vi "Build New Ballard ARINC 429 Custom Device.vi"(7 "Base System Definition File":path=path "Support/Base.nivssdf", 10 "Hardware Configuration File":path=path "Support/Multichannel Tx and Rx HW.xml", 11 "Output System Definition File":path=path "Support/Scripted Ballard ARINC 429.nivssdf") -> (3 "Ballard ARINC 429 System Definition":path)   [LabVIEW 2020]
doc: "Overview: Demonstrates using the Ballard ARINC 429 scripting API to configure the custom device by building from configuration clusters. \n\nInstructions:\n1. Specify the Hardware Configuration File. The hardware configuration file must be consistent with the schema installed by the Ballard hardware driver at C:\\Program Files (x86)\\Astronics Ballard Technology LabVIEW Driver\\Help\\index.html. The hardware configuration file must also be consistent with the configuration in this example VI.\n2. (VeriStand) Optionally, you may open the Output System Definition File in VeriStand, configure the Target, and deploy the scripted system definition to perform avionics bus communications with Ballard ARINC 429 hardware."
uses:
  Ballard ARINC 429 Scripting Examples.lvlib
  <vilib>/addons/VeriStand Custom Device Scripting APIs/Ballard ARINC 429/Scripting/Ballard/Ballard ARINC 429 Scripting.lvlib
  <vilib>/addons/VeriStand Custom Device Scripting APIs/Ballard ARINC 429/Shared/Direction.ctl
  <vilib>/addons/VeriStand Custom Device Scripting APIs/Ballard ARINC 429/Shared/Ballard ARINC 429 Shared.lvlib
  <vilib>/addons/VeriStand Custom Device Scripting APIs/Ballard ARINC 429/Shared/SDI.ctl
  <vilib>/addons/VeriStand Custom Device Scripting APIs/Ballard ARINC 429/Shared/Transfer Type.ctl
  <vilib>/NI/NI VeriStand Encoding and Decoding/Encoding.ctl
  <vilib>/NI/NI VeriStand Encoding and Decoding/Encoding and Decoding.lvlib
  <vilib>/addons/VeriStand Custom Device Scripting APIs/Ballard ARINC 429/Shared/Parameter Definition.ctl
  NationalInstruments.VeriStand.SystemDefinitionAPI
  <vilib>/addons/VeriStand Custom Device Scripting APIs/Ballard ARINC 429/Shared/Initialization Method.ctl
  <vilib>/addons/VeriStand Custom Device Scripting APIs/Ballard ARINC 429/Shared/Device Parameters.ctl
panel:
  # "Overview: Demonstrates using the Ballard ARINC 429 scripting API to configure the custom device by building from configuration clusters. \n\nInstructions:\n1. Specify the Hardware Configuration File. The hardware configuration file must be consistent with the schema installed by the Ballard hardware driver at C:\\Program Files (x86)\\Astronics Ballard Technology LabVIEW Driver\\Help\\index.html. The hardware configuration file must also be consistent with the configuration in this example VI.\n2. (VeriStand) Optionally, you may open the Output System Definition File in VeriStand, configure the Target, and deploy the scripted system definition to perform avionics bus communications with Ballard ARINC 429 hardware."
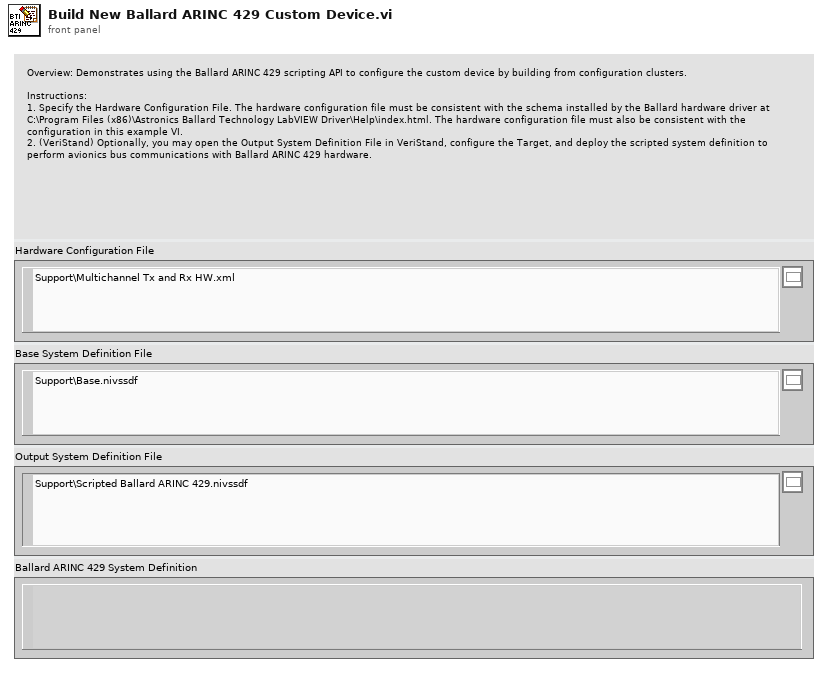
[diagram p1: front panel]
types:
  T1 = typedef "Ballard ARINC 429 Shared.lvlib/Device Parameters.ctl" = cluster{"initialization method":T2, "card number":i32, "PXI slot number":i32, "core number":i32, "core serial number":i32}
  T2 = typedef "Ballard ARINC 429 Shared.lvlib/Initialization Method.ctl" = enum16{"PXI Slot Number", "Card Number", "Core Serial Number"}
  T3 = cluster{"name":string, "unit":string, "default value":dbl}[]
  T4 = typedef "Ballard ARINC 429 Shared.lvlib/Parameter Definition.ctl" = cluster{"start index":i32, "size":i32, "encoding":T5, "signed":bool, "scale multiplier":dbl, "scale offset":dbl}
  T5 = typedef "Encoding and Decoding.lvlib/Encoding.ctl" = enum16{"BNR", "BCD", "Discrete"}
  T6 = typedef "Ballard ARINC 429 Shared.lvlib/Direction.ctl" = enum16{"Rx", "Tx"}
  T7 = typedef "Ballard ARINC 429 Shared.lvlib/Transfer Type.ctl" = enum16{"Scheduled", "Acyclic", "Block", "Strobe"}
  T8 = typedef "Ballard ARINC 429 Shared.lvlib/SDI.ctl" = i32
  T9 = typedef "Custom Device API.lvlib/Custom Device Item Ref.ctl" = u64
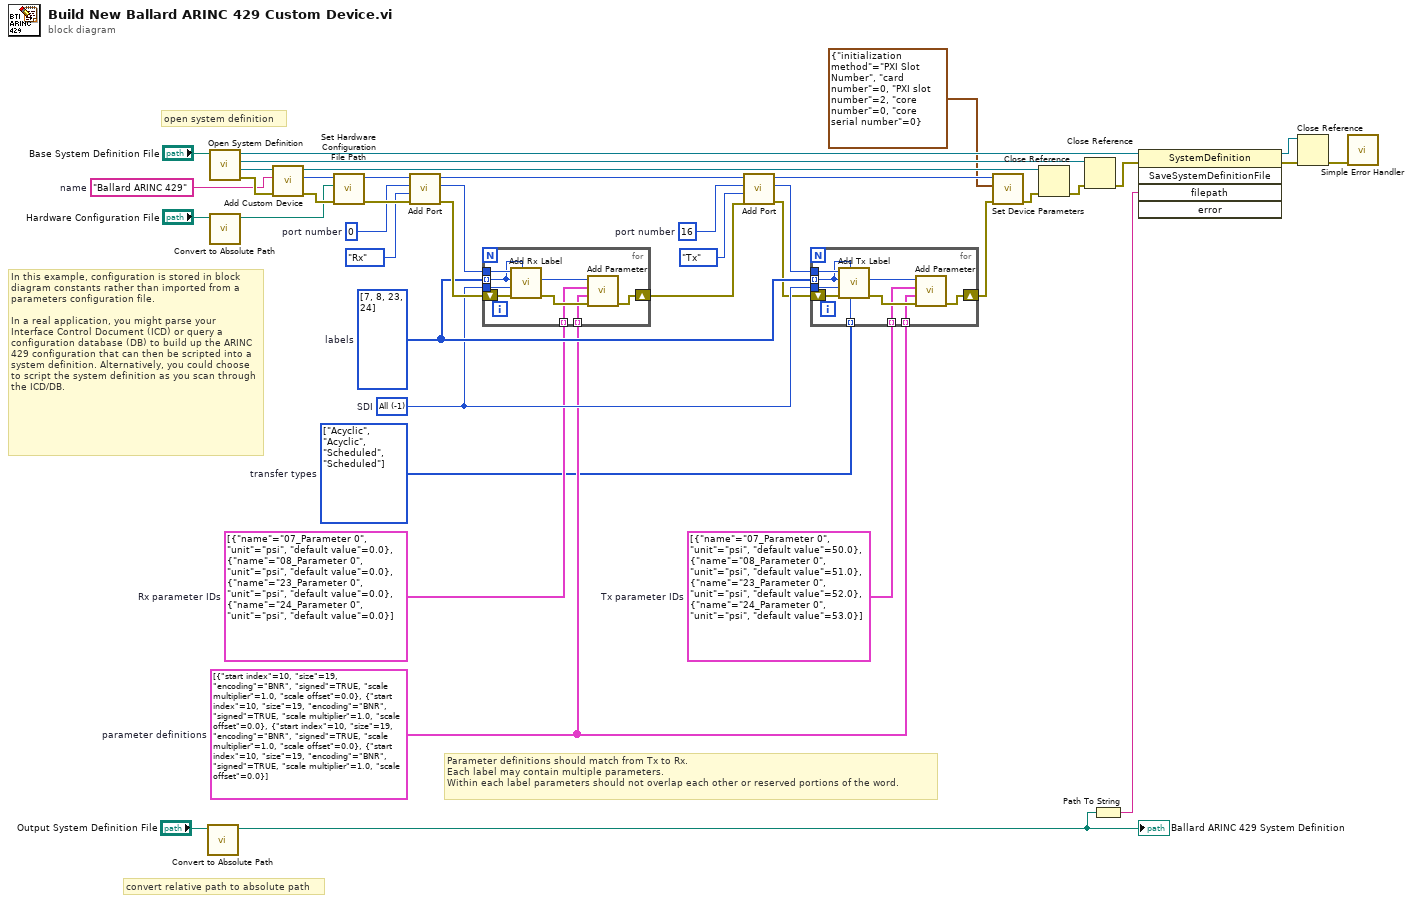
[diagram p0: block diagram]
diagram:
  w6 = T3 [{"name"="07_Parameter 0", "unit"="psi", "default value"=50.0}, {"name"="08_Parameter 0", "unit"="psi", "default value"=51.0}, {"name"="23_Parameter 0", "unit"="psi", "default value"=52.0}, {"name"="24_Parameter 0", "unit"="psi", "default value"=53.0}]  # Tx parameter IDs
  w8 = T4[] [{"start index"=10, "size"=19, "encoding"=enum."BNR", "signed"=TRUE, "scale multiplier"=1.0, "scale offset"=0.0}, {"start index"=10, "size"=19, "encoding"=enum."BNR", "signed"=TRUE, "scale multiplier"=1.0, "scale offset"=0.0}, {"start index"=10, "size"=19, "encoding"=enum."BNR", "signed"=TRUE, "scale multiplier"=1.0, "scale offset"=0.0}, {"start index"=10, "size"=19, "encoding"=enum."BNR", "signed"=TRUE, "scale multiplier"=1.0, "scale offset"=0.0}]  # parameter definitions
  w9 = T3 [{"name"="07_Parameter 0", "unit"="psi", "default value"=0.0}, {"name"="08_Parameter 0", "unit"="psi", "default value"=0.0}, {"name"="23_Parameter 0", "unit"="psi", "default value"=0.0}, {"name"="24_Parameter 0", "unit"="psi", "default value"=0.0}]  # Rx parameter IDs
  w17 = u16 16  # port number
  w7 = T7[] [enum."Acyclic", enum."Acyclic", enum."Scheduled", enum."Scheduled"] items=["Scheduled", "Acyclic", "Block", "Strobe"]  # transfer types
  w11 = T8 -1 items=["All"=-1, "0 (b00)"=0, "1 (b01)"=1, "2 (b10)"=2, "3 (b11)"=3]  # SDI
  w12 = u32[] [7, 8, 23, 24]  # labels
  w19 = u16 0  # port number
  w27 = "Ballard ARINC 429"  # name
  # "open system definition"
  # "convert relative path to absolute path"
  # "Parameter definitions should match from Tx to Rx.\nEach label may contain multiple parameters.\nWithin each label parameters should not overlap each other or reserved portions of the word."
  # "In this example, configuration is stored in block diagram constants rather than imported from a parameters configuration file.\n\nIn a real application, you might parse your Interface Control Document (ICD) or query a configuration database (DB) to build up the ARINC 429 configuration that can then be scripted into a system definition. Alternatively, you could choose to script the system definition as you scan through the ICD/DB."
  # "8."
  n1 = call "Convert to Absolute Path.vi"("system definition file"="Output System Definition File") -> ("absolute path"=w5:path)  [unwired: 10 in]
  "Ballard ARINC 429 System Definition" <- w5
  n2 = call "Open System Definition.vi"("system definition file"="Base System Definition File") -> ("error out"=w30:errorcluster, "target"=w29:refnum<k24>, "root"=w33:refnum<k24>, "system definition"=w34:refnum<k24>)  [unwired: 7 in]
  n3 = call "Convert to Absolute Path.vi"("system definition file"="Hardware Configuration File") -> ("absolute path"=w24:path)  [unwired: 10 in]
  n4 = call <vilib>:"Add Custom Device.vi"("error in"=w30, "name"=w27, "target in"=w29) -> ("error out"=w25:errorcluster, "Ballard ARINC 429 custom device"=w26:T9, "target out"=w28:refnum<k24>)  [unwired: 6 in]
  n5 = call <vilib>:"Set Hardware Configuration File Path.vi"("error in"=w25, "hardware configuration file path"=w24, "Ballard ARINC 429 custom device in"=w26) -> ("error out"=w22:errorcluster, "Ballard ARINC 429 custom device out"=w23:T9)  [unwired: 7 in]
  n6 = call <vilib>:"Add Port.vi"("error in"=w22, "direction"=Direction."Rx", "port number"=w19, "Ballard ARINC 429 custom device in"=w23) -> ("error out"=w20:errorcluster, "port"=w21:T9, "Ballard ARINC 429 custom device out"=w15:T9)  [unwired: 5 in]
  n7 = for {
    tunnel: w21 -> [w50]
    tunnel: w11 -> [w48]
    shift-right: [w45] -> w14
    shift-left: w20 -> [w49]
    tunnel: w12 -> [w42] mode=indexing
    tunnel: w9 -> [w44] mode=indexing
    tunnel: w8 -> [w43] mode=indexing
    n8 = call <vilib>:"Add Rx Label.vi"("label (Display)"=w42, "error in"=w49, "SDI value"=w48, "label (Dec)"=w42, "port in"=w50) -> ("error out"=w46:errorcluster, "label"=w47:T9)  [unwired: 4 in, 1 out]
    n9 = call <vilib>:"Add Parameter.vi"("error in"=w46, "parameter encoding"=w43, "parameter definition"=w44, "label in"=w47) -> ("error out"=w45:errorcluster)  [unwired: 5 in, 2 out]
  }
  n10 = call <vilib>:"Add Port.vi"("error in"=w14, "direction"=Direction."Tx", "port number"=w17, "Ballard ARINC 429 custom device in"=w15) -> ("error out"=w10:errorcluster, "port"=w13:T9, "Ballard ARINC 429 custom device out"=w4:T9)  [unwired: 5 in]
  n11 = for {
    tunnel: w13 -> [w60]
    tunnel: w11 -> [w58]
    shift-right: [w55] -> w3
    shift-left: w10 -> [w59]
    tunnel: w12 -> [w51] mode=indexing
    tunnel: w6 -> [w54] mode=indexing
    tunnel: w8 -> [w53] mode=indexing
    tunnel: w7 -> [w52] mode=indexing
    n12 = call <vilib>:"Add Tx Label.vi"("transfer type"=w52, "label (Display)"=w51, "error in"=w59, "SDI value"=w58, "label (Dec)"=w51, "port in"=w60) -> ("error out"=w56:errorcluster, "label"=w57:T9)  [unwired: 3 in, 1 out]
    n13 = call <vilib>:"Add Parameter.vi"("error in"=w56, "parameter encoding"=w53, "parameter definition"=w54, "label in"=w57) -> ("error out"=w55:errorcluster)  [unwired: 5 in, 2 out]
  }
  n14 = call <vilib>:"Set Device Parameters.vi"("error in"=w3, "device parameters"=T1 {"initialization method"=enum."PXI Slot Number", "card number"=0, "PXI slot number"=2, "core number"=0, "core serial number"=0}, "Ballard ARINC 429 custom device in"=w4) -> ("error out"=w2:errorcluster)  [unwired: 7 in, 1 out]
  n15 = Close Reference(reference=w28, error in (no error)=w2) -> (error out=w32:errorcluster)
  n16 = Close Reference(reference=w33, error in (no error)=w32) -> (error out=w37:errorcluster)
  n17 = Path To String(path=w5) -> (string=w40:string)
  n18 = invoke class="SystemDefinition" method="SaveSystemDefinitionFile"(reference=w34, error in=w37, "filepath"=w40) -> (reference out=w38:refnum<k24>, error out=w39:errorcluster)  [unwired: 2 in, 3 out]
  n19 = Close Reference(reference=w38, error in (no error)=w39) -> (error out=w36:errorcluster)
  n20 = call <vilib>:"Simple Error Handler.vi"("error in (no error)"=w36) -> ()  [unwired: 1 in, 8 out]
